vi "Test Plant First Order Step B.vi"(8 "error in":errorcluster) -> (0 "error out":errorcluster)   [LabVIEW 2026]
doc: "Caraya test of Plant First Order Step.vi: decay, chaining, steady state, dt 0 (FOS-5..10)."
uses:
  <vilib>/addons/_JKI Toolkits/Caraya/classes/Test/Test.lvclass
  <vilib>/addons/_JKI Toolkits/Caraya/classes/Assert/Assert.lvclass
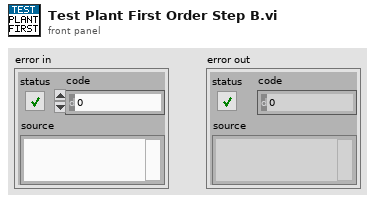
[diagram p1: front panel]
types:
  T1 = cluster{"pressure_sp_bar":dbl, "flow_sp_lpm":dbl, "displacement_sp_mm":dbl}
  T2 = cluster{"pressure_bar":dbl, "flow_lpm":dbl, "displacement_mm":dbl, "timestamp_ms":dbl}
  T3 = typedef "Plant Feedback.ctl" = cluster{"pressure_bar":dbl, "flow_lpm":dbl, "displacement_mm":dbl, "timestamp_ms":dbl}
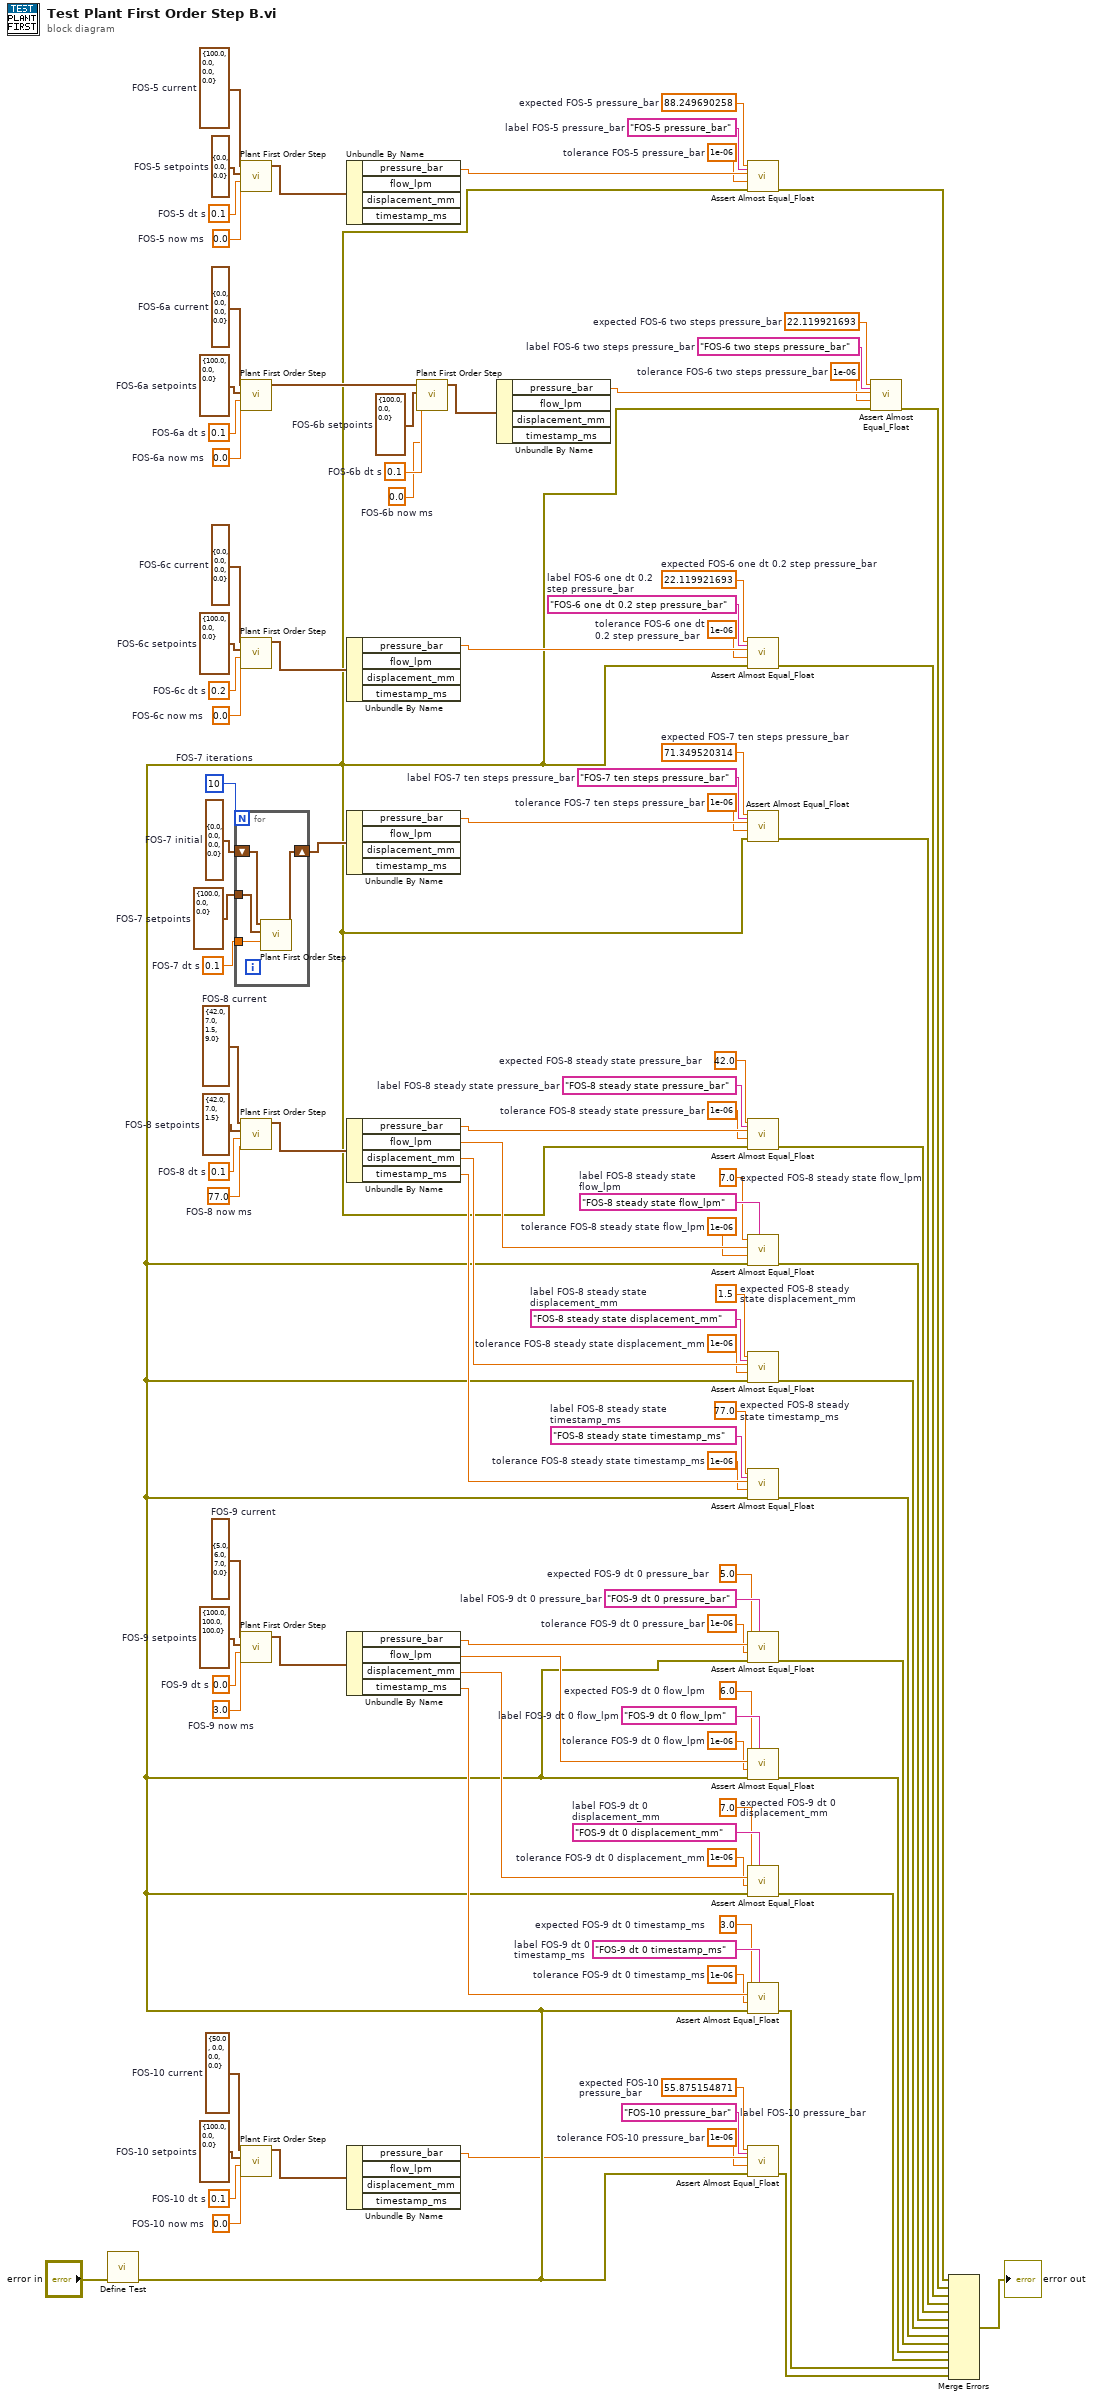
[diagram p0: block diagram]
diagram:
  w19 = "FOS-10 pressure_bar"  # label FOS-10 pressure_bar
  w15 = 1e-06  # tolerance FOS-10 pressure_bar
  w17 = 55.875154871  # expected FOS-10 pressure_bar
  w21 = 0.0  # FOS-10 now ms
  w22 = 0.1  # FOS-10 dt s
  w23 = T1 {"pressure_sp_bar"=100.0, "flow_sp_lpm"=0.0, "displacement_sp_mm"=0.0}  # FOS-10 setpoints
  w24 = T2 {"pressure_bar"=50.0, "flow_lpm"=0.0, "displacement_mm"=0.0, "timestamp_ms"=0.0}  # FOS-10 current
  w28 = "FOS-9 dt 0 timestamp_ms"  # label FOS-9 dt 0 timestamp_ms
  w25 = 1e-06  # tolerance FOS-9 dt 0 timestamp_ms
  w27 = 3.0  # expected FOS-9 dt 0 timestamp_ms
  w32 = "FOS-9 dt 0 displacement_mm"  # label FOS-9 dt 0 displacement_mm
  w29 = 1e-06  # tolerance FOS-9 dt 0 displacement_mm
  w31 = 7.0  # expected FOS-9 dt 0 displacement_mm
  w36 = "FOS-9 dt 0 flow_lpm"  # label FOS-9 dt 0 flow_lpm
  w33 = 1e-06  # tolerance FOS-9 dt 0 flow_lpm
  w35 = 6.0  # expected FOS-9 dt 0 flow_lpm
  w40 = "FOS-9 dt 0 pressure_bar"  # label FOS-9 dt 0 pressure_bar
  w37 = 1e-06  # tolerance FOS-9 dt 0 pressure_bar
  w39 = 5.0  # expected FOS-9 dt 0 pressure_bar
  w42 = 3.0  # FOS-9 now ms
  w43 = 0.0  # FOS-9 dt s
  w44 = T1 {"pressure_sp_bar"=100.0, "flow_sp_lpm"=100.0, "displacement_sp_mm"=100.0}  # FOS-9 setpoints
  w45 = T2 {"pressure_bar"=5.0, "flow_lpm"=6.0, "displacement_mm"=7.0, "timestamp_ms"=0.0}  # FOS-9 current
  w49 = "FOS-8 steady state timestamp_ms"  # label FOS-8 steady state timestamp_ms
  w46 = 1e-06  # tolerance FOS-8 steady state timestamp_ms
  w48 = 77.0  # expected FOS-8 steady state timestamp_ms
  w53 = "FOS-8 steady state displacement_mm"  # label FOS-8 steady state displacement_mm
  w50 = 1e-06  # tolerance FOS-8 steady state displacement_mm
  w52 = 1.5  # expected FOS-8 steady state displacement_mm
  w57 = "FOS-8 steady state flow_lpm"  # label FOS-8 steady state flow_lpm
  w54 = 1e-06  # tolerance FOS-8 steady state flow_lpm
  w56 = 7.0  # expected FOS-8 steady state flow_lpm
  w61 = "FOS-8 steady state pressure_bar"  # label FOS-8 steady state pressure_bar
  w58 = 1e-06  # tolerance FOS-8 steady state pressure_bar
  w60 = 42.0  # expected FOS-8 steady state pressure_bar
  w63 = 77.0  # FOS-8 now ms
  w64 = 0.1  # FOS-8 dt s
  w65 = T1 {"pressure_sp_bar"=42.0, "flow_sp_lpm"=7.0, "displacement_sp_mm"=1.5}  # FOS-8 setpoints
  w66 = T2 {"pressure_bar"=42.0, "flow_lpm"=7.0, "displacement_mm"=1.5, "timestamp_ms"=9.0}  # FOS-8 current
  w70 = "FOS-7 ten steps pressure_bar"  # label FOS-7 ten steps pressure_bar
  w67 = 1e-06  # tolerance FOS-7 ten steps pressure_bar
  w69 = 71.349520314  # expected FOS-7 ten steps pressure_bar
  w74 = 0.1  # FOS-7 dt s
  w75 = T1 {"pressure_sp_bar"=100.0, "flow_sp_lpm"=0.0, "displacement_sp_mm"=0.0}  # FOS-7 setpoints
  w72 = 10  # FOS-7 iterations
  w73 = T2 {"pressure_bar"=0.0, "flow_lpm"=0.0, "displacement_mm"=0.0, "timestamp_ms"=0.0}  # FOS-7 initial
  w79 = "FOS-6 one dt 0.2 step pressure_bar"  # label FOS-6 one dt 0.2 step pressure_bar
  w76 = 1e-06  # tolerance FOS-6 one dt 0.2 step pressure_bar
  w78 = 22.119921693  # expected FOS-6 one dt 0.2 step pressure_bar
  w81 = 0.0  # FOS-6c now ms
  w82 = 0.2  # FOS-6c dt s
  w83 = T1 {"pressure_sp_bar"=100.0, "flow_sp_lpm"=0.0, "displacement_sp_mm"=0.0}  # FOS-6c setpoints
  w84 = T2 {"pressure_bar"=0.0, "flow_lpm"=0.0, "displacement_mm"=0.0, "timestamp_ms"=0.0}  # FOS-6c current
  w88 = "FOS-6 two steps pressure_bar"  # label FOS-6 two steps pressure_bar
  w85 = 1e-06  # tolerance FOS-6 two steps pressure_bar
  w87 = 22.119921693  # expected FOS-6 two steps pressure_bar
  w90 = 0.0  # FOS-6b now ms
  w91 = 0.1  # FOS-6b dt s
  w92 = T1 {"pressure_sp_bar"=100.0, "flow_sp_lpm"=0.0, "displacement_sp_mm"=0.0}  # FOS-6b setpoints
  w94 = 0.0  # FOS-6a now ms
  w95 = 0.1  # FOS-6a dt s
  w96 = T1 {"pressure_sp_bar"=100.0, "flow_sp_lpm"=0.0, "displacement_sp_mm"=0.0}  # FOS-6a setpoints
  w97 = T2 {"pressure_bar"=0.0, "flow_lpm"=0.0, "displacement_mm"=0.0, "timestamp_ms"=0.0}  # FOS-6a current
  w101 = "FOS-5 pressure_bar"  # label FOS-5 pressure_bar
  w98 = 1e-06  # tolerance FOS-5 pressure_bar
  w100 = 88.249690258  # expected FOS-5 pressure_bar
  w103 = 0.0  # FOS-5 now ms
  w104 = 0.1  # FOS-5 dt s
  w105 = T1 {"pressure_sp_bar"=0.0, "flow_sp_lpm"=0.0, "displacement_sp_mm"=0.0}  # FOS-5 setpoints
  w106 = T2 {"pressure_bar"=100.0, "flow_lpm"=0.0, "displacement_mm"=0.0, "timestamp_ms"=0.0}  # FOS-5 current
  n1 = call <vilib>:"Define Test.vi"("error in (no error)"="error in") -> ("error out"=w18:errorcluster)  [unwired: 9 in, 1 out]
  n2 = for {
    N: w72 -> [_]
    tunnel: w75 -> [w111]
    tunnel: w74 -> [w110]
    shift-right: [w109] -> w71
    shift-left: w73 -> [w108]
    n3 = call "Plant First Order Step.vi"("dt s"=w110, "Plant Setpoints"=w111, "current Plant Feedback"=w108) -> ("new Plant Feedback"=w109:T3)  [unwired: 8 in]
  }
  n4 = call "Plant First Order Step.vi"("now ms"=w103, "dt s"=w104, "Plant Setpoints"=w105, "current Plant Feedback"=w106) -> ("new Plant Feedback"=w102:T3)  [unwired: 7 in]
  n5 = call "Plant First Order Step.vi"("now ms"=w94, "dt s"=w95, "Plant Setpoints"=w96, "current Plant Feedback"=w97) -> ("new Plant Feedback"=w93:T3)  [unwired: 7 in]
  n6 = call "Plant First Order Step.vi"("now ms"=w81, "dt s"=w82, "Plant Setpoints"=w83, "current Plant Feedback"=w84) -> ("new Plant Feedback"=w80:T3)  [unwired: 7 in]
  n7 = call "Plant First Order Step.vi"("now ms"=w63, "dt s"=w64, "Plant Setpoints"=w65, "current Plant Feedback"=w66) -> ("new Plant Feedback"=w62:T3)  [unwired: 7 in]
  n8 = call "Plant First Order Step.vi"("now ms"=w42, "dt s"=w43, "Plant Setpoints"=w44, "current Plant Feedback"=w45) -> ("new Plant Feedback"=w41:T3)  [unwired: 7 in]
  n9 = call "Plant First Order Step.vi"("now ms"=w21, "dt s"=w22, "Plant Setpoints"=w23, "current Plant Feedback"=w24) -> ("new Plant Feedback"=w20:T3)  [unwired: 7 in]
  n10 = Unbundle By Name(w102) -> ("pressure_bar"=w99:dbl)  [unwired: 3 out]
  n11 = Unbundle By Name(w80) -> ("pressure_bar"=w77:dbl)  [unwired: 3 out]
  n12 = Unbundle By Name(w71) -> ("pressure_bar"=w68:dbl)  [unwired: 3 out]
  n13 = Unbundle By Name(w62) -> ("pressure_bar"=w59:dbl, "flow_lpm"=w55:dbl, "displacement_mm"=w51:dbl, "timestamp_ms"=w47:dbl)
  n14 = Unbundle By Name(w41) -> ("pressure_bar"=w38:dbl, "flow_lpm"=w34:dbl, "displacement_mm"=w30:dbl, "timestamp_ms"=w26:dbl)
  n15 = Unbundle By Name(w20) -> ("pressure_bar"=w16:dbl)  [unwired: 3 out]
  n16 = call "Plant First Order Step.vi"("now ms"=w90, "dt s"=w91, "Plant Setpoints"=w92, "current Plant Feedback"=w93) -> ("new Plant Feedback"=w89:T3)  [unwired: 7 in]
  n17 = Unbundle By Name(w89) -> ("pressure_bar"=w86:dbl)  [unwired: 3 out]
  n18 = call <vilib>:"Assert Almost Equal_Float.vi"("Label"=w101, "error in (no error)"=w18, "Tolerance"=w98, "Actual"=w99, "Expected"=w100) -> ("error out"=w14:errorcluster)  [unwired: 5 in, 1 out]
  n19 = call <vilib>:"Assert Almost Equal_Float.vi"("Label"=w79, "error in (no error)"=w18, "Tolerance"=w76, "Actual"=w77, "Expected"=w78) -> ("error out"=w12:errorcluster)  [unwired: 5 in, 1 out]
  n20 = call <vilib>:"Assert Almost Equal_Float.vi"("Label"=w70, "error in (no error)"=w18, "Tolerance"=w67, "Actual"=w68, "Expected"=w69) -> ("error out"=w11:errorcluster)  [unwired: 5 in, 1 out]
  n21 = call <vilib>:"Assert Almost Equal_Float.vi"("Label"=w61, "error in (no error)"=w18, "Tolerance"=w58, "Actual"=w59, "Expected"=w60) -> ("error out"=w10:errorcluster)  [unwired: 5 in, 1 out]
  n22 = call <vilib>:"Assert Almost Equal_Float.vi"("Label"=w57, "error in (no error)"=w18, "Tolerance"=w54, "Actual"=w55, "Expected"=w56) -> ("error out"=w9:errorcluster)  [unwired: 5 in, 1 out]
  n23 = call <vilib>:"Assert Almost Equal_Float.vi"("Label"=w53, "error in (no error)"=w18, "Tolerance"=w50, "Actual"=w51, "Expected"=w52) -> ("error out"=w8:errorcluster)  [unwired: 5 in, 1 out]
  n24 = call <vilib>:"Assert Almost Equal_Float.vi"("Label"=w49, "error in (no error)"=w18, "Tolerance"=w46, "Actual"=w47, "Expected"=w48) -> ("error out"=w7:errorcluster)  [unwired: 5 in, 1 out]
  n25 = call <vilib>:"Assert Almost Equal_Float.vi"("Label"=w40, "error in (no error)"=w18, "Tolerance"=w37, "Actual"=w38, "Expected"=w39) -> ("error out"=w6:errorcluster)  [unwired: 5 in, 1 out]
  n26 = call <vilib>:"Assert Almost Equal_Float.vi"("Label"=w36, "error in (no error)"=w18, "Tolerance"=w33, "Actual"=w34, "Expected"=w35) -> ("error out"=w5:errorcluster)  [unwired: 5 in, 1 out]
  n27 = call <vilib>:"Assert Almost Equal_Float.vi"("Label"=w32, "error in (no error)"=w18, "Tolerance"=w29, "Actual"=w30, "Expected"=w31) -> ("error out"=w4:errorcluster)  [unwired: 5 in, 1 out]
  n28 = call <vilib>:"Assert Almost Equal_Float.vi"("Label"=w28, "error in (no error)"=w18, "Tolerance"=w25, "Actual"=w26, "Expected"=w27) -> ("error out"=w3:errorcluster)  [unwired: 5 in, 1 out]
  n29 = call <vilib>:"Assert Almost Equal_Float.vi"("Label"=w19, "error in (no error)"=w18, "Tolerance"=w15, "Actual"=w16, "Expected"=w17) -> ("error out"=w2:errorcluster)  [unwired: 5 in, 1 out]
  n30 = call <vilib>:"Assert Almost Equal_Float.vi"("Label"=w88, "error in (no error)"=w18, "Tolerance"=w85, "Actual"=w86, "Expected"=w87) -> ("error out"=w13:errorcluster)  [unwired: 5 in, 1 out]
  n31 = Merge Errors(w14, w13, w12, w11, w10, w9, w8, w7, w6, w5, w4, w3, w2) -> (→"error out":errorcluster)
